vi "包装Main.vi"() -> ()   [LabVIEW 2024]
panel:
  in  "重复包装":dbl
  out "客户码数量":i16
  out "上线码数量":i16
  in  "直接打箱码，慎用！":bool
  out "烘干":bool
  out "烘干工位号":string
  out "重复包装":bool
  in  "切换":bool=TRUE
  in  "扫码结果（流水码）-仅查询":string
  out "清洗":bool
  out "干检":bool
  out "氦检":bool
  out "字符串":string
  out "数值":i32
  out "长度":i32
  out "当前箱码":string
  in  "箱码序号":dbl format="%0#3_5f"
  out "包装完成":bool
  in  "包装累计":dbl
  in  "包装过程":dbl
  in  "扫码结果（客户码）-包装用":string
  in  "设定包装数量":dbl
  in  "装箱产品":string[](array[string])
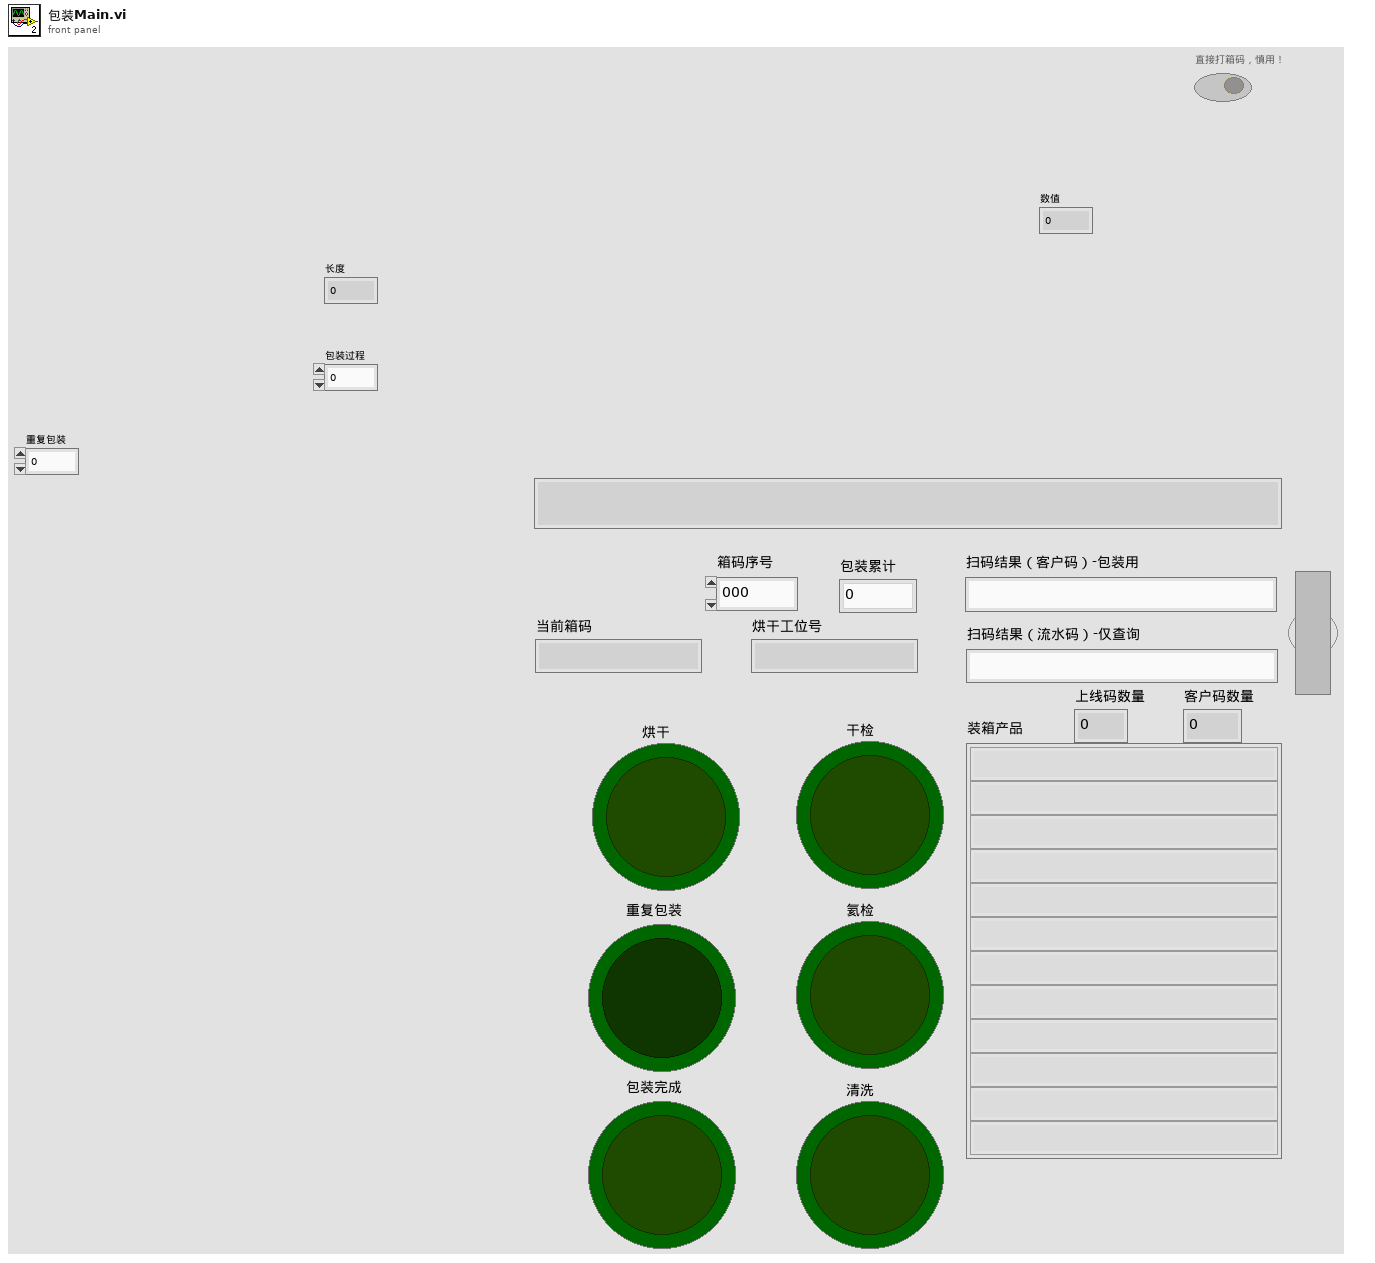
[diagram p1: front panel]
types:
  T1 = enum16{"Standard", "Buffered", "CRLF", "Immediate"}
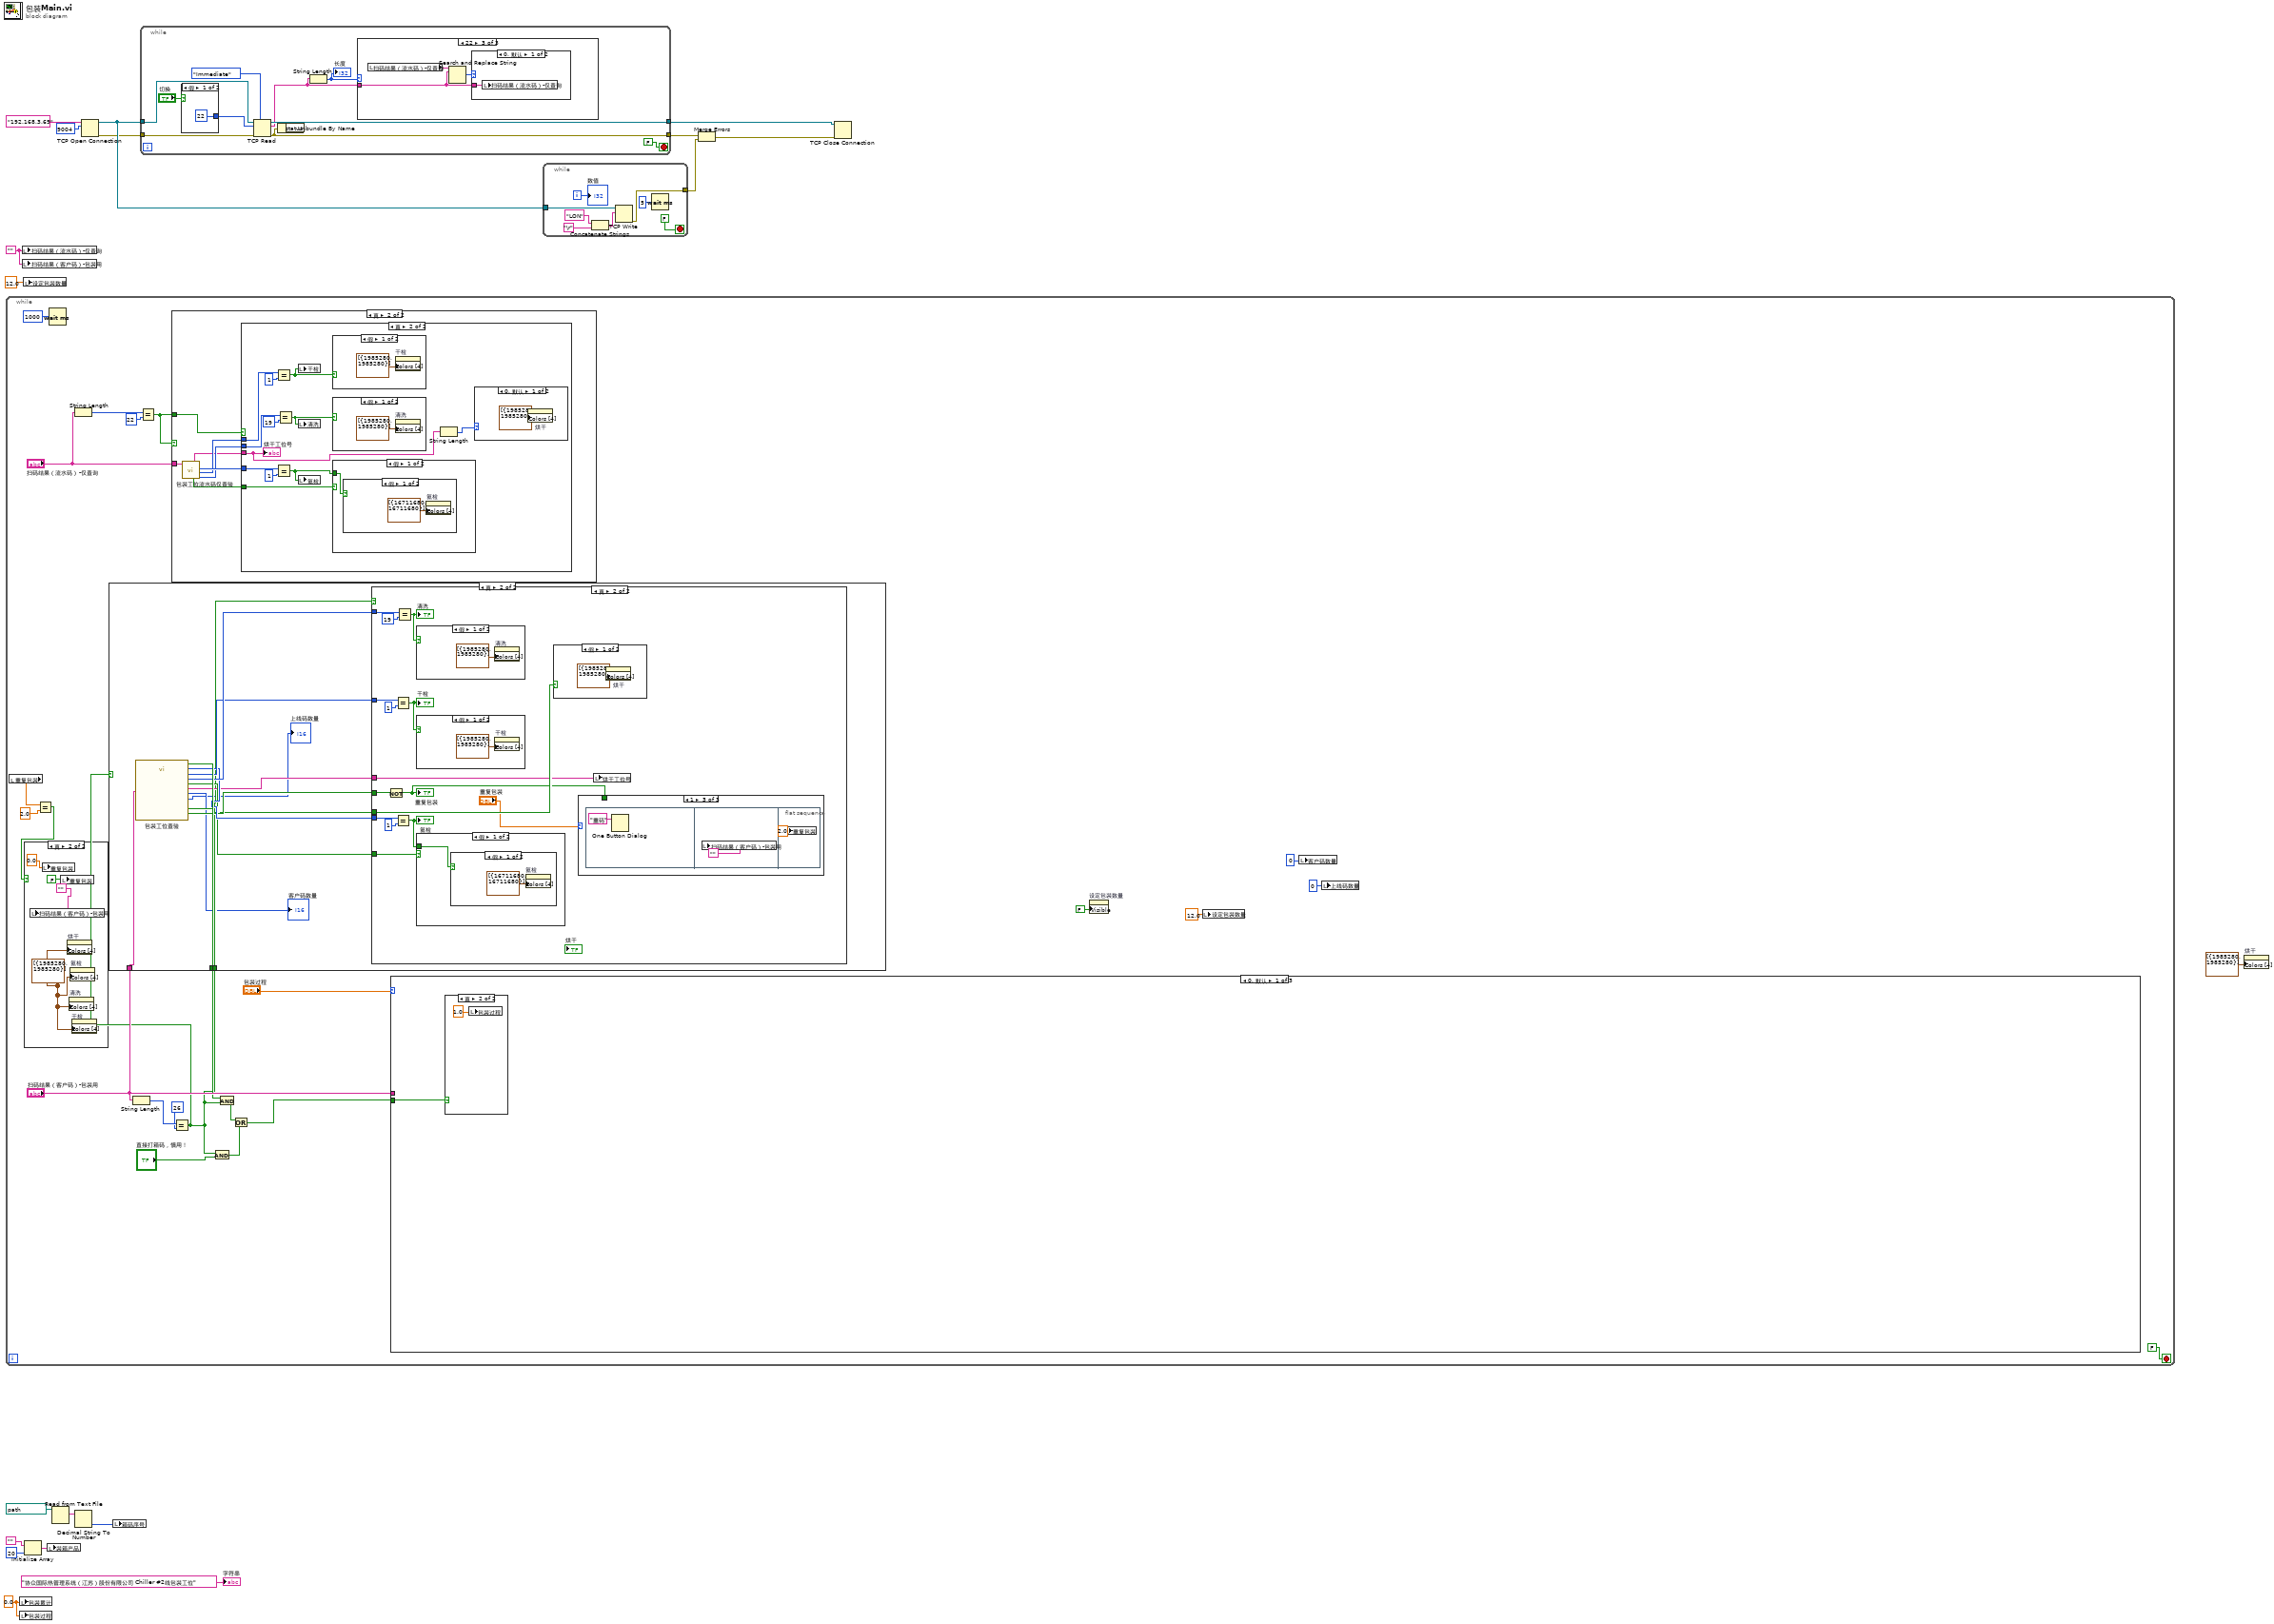
[diagram p0: block diagram]
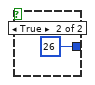
[diagram p2: hidden frame]
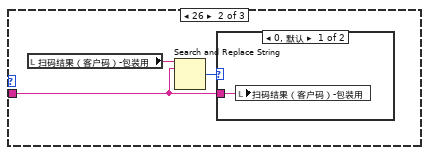
[diagram p4: hidden frame]
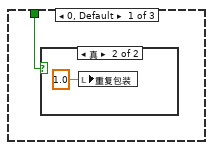
[diagram p10: hidden frame]
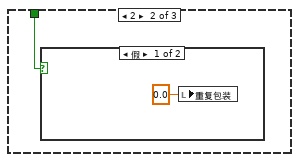
[diagram p12: hidden frame]
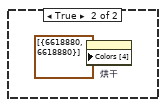
[diagram p14: hidden frame]
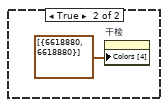
[diagram p15: hidden frame]
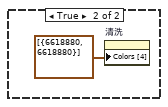
[diagram p16: hidden frame]
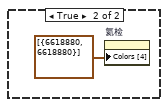
[diagram p17: hidden frame]
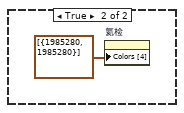
[diagram p18: hidden frame]
diagram:
  w2 = ""
  w19 = 0.0 ("包装过程")
  n1 = while {
    stop <- FALSE stop-if-true
    n2 = local read "重复包装"() -> (w22:dbl)
    n3 = Equal?(x=w22, y=2.0) -> (x = y?=w20:bool)
    n4 = case shown="真" w20 {
      frame False {
      }
      frame True {
        w44 = cluster{u32, u32}[] [{1985280, 1985280}] ("颜色[4]")
        n5 = local write "扫码结果（客户码）-包装用"("") -> ()
        n6 = local write "重复包装"(0.0 ("重复包装")) -> ()
        n7 = local write "重复包装"(FALSE ("重复包装")) -> ()
        n8 = property on="烘干" class="Bool (严格)"("Colors [4]"=w44) -> ()  [unwired: 2 in, 2 out]
        n9 = property on="清洗" class="Bool (严格)"("Colors [4]"=w44) -> ()  [unwired: 2 in, 2 out]
        n10 = property on="氦检" class="Bool (严格)"("Colors [4]"=w44) -> ()  [unwired: 2 in, 2 out]
        n11 = property on="干检" class="Bool (严格)"("Colors [4]"=w44) -> ()  [unwired: 2 in, 2 out]
      }
    }
    n12 = Wait (ms)(milliseconds to wait=u32 1000 ("等待时间（毫秒）")) -> ()  [unwired: 1 out]
    n13 = String Length(string="扫码结果（流水码）-仅查询") -> (length=w34:i32)
    n14 = String Length(string="扫码结果（客户码）-包装用") -> (length=w40:i32)
    n15 = Equal?(x=w34, y=22) -> (x = y?=w28:bool)
    n16 = case shown="真" w28 {
      tunnel: "扫码结果（流水码）-仅查询" -> [_ w97]
      tunnel: w28 -> [_ w96]
      frame False {
      }
      frame True {
        n17 = call "包装工位流水码仅查验.vi"("流水码编号"=w97) -> ("长度"=w93:i32, "干检OK"=w94:i32, "氦检OK"=w95:i32, "没氦检"=w92:bool, "烘干工位号"=w91:string)  [unwired: 5 in, 1 out]
        n18 = case shown="真" w96 {
          tunnel: w95 -> [_ w106]
          tunnel: w94 -> [_ w105]
          tunnel: w93 -> [_ w104]
          tunnel: w92 -> [_ w103]
          tunnel: w91 -> [_ w99]
          frame False {
          }
          frame True {
            n19 = Equal?(x=w105, y=1) -> (x = y?=w100:bool)
            n20 = Equal?(x=w106, y=1) -> (x = y?=w102:bool)
            n21 = Equal?(x=w104, y=19) -> (x = y?=w101:bool)
            n22 = local write "干检"(w100) -> ()
            n23 = local write "清洗"(w101) -> ()
            n24 = local write "氦检"(w102) -> ()
            n25 = case shown="假" w100 {
              frame False {
                n26 = property on="干检" class="Bool (严格)"("Colors [4]"=cluster{u32, u32}[] [{1985280, 1985280}] ("颜色[4]")) -> ()  [unwired: 2 in, 2 out]
              }
              frame True {
                n27 = property on="干检" class="Bool (严格)"("Colors [4]"=cluster{u32, u32}[] [{6618880, 6618880}] ("颜色[4]")) -> ()  [unwired: 2 in, 2 out]
              }
            }
            n28 = case shown="假" w101 {
              frame False {
                n29 = property on="清洗" class="Bool (严格)"("Colors [4]"=cluster{u32, u32}[] [{1985280, 1985280}] ("颜色[4]")) -> ()  [unwired: 2 in, 2 out]
              }
              frame True {
                n30 = property on="清洗" class="Bool (严格)"("Colors [4]"=cluster{u32, u32}[] [{6618880, 6618880}] ("颜色[4]")) -> ()  [unwired: 2 in, 2 out]
              }
            }
            n31 = case shown="假" w103 {
              tunnel: w102 -> [w116 _]
              frame False {
                n32 = case shown="假" w116 {
                  frame False {
                    n33 = property on="氦检" class="Bool (严格)"("Colors [4]"=cluster{u32, u32}[] [{16711680, 16711680}] ("颜色[4]")) -> ()  [unwired: 2 in, 2 out]
                  }
                  frame True {
                    n34 = property on="氦检" class="Bool (严格)"("Colors [4]"=cluster{u32, u32}[] [{6618880, 6618880}] ("颜色[4]")) -> ()  [unwired: 2 in, 2 out]
                  }
                }
              }
              frame True {
                n35 = property on="氦检" class="Bool (严格)"("Colors [4]"=cluster{u32, u32}[] [{1985280, 1985280}] ("颜色[4]")) -> ()  [unwired: 2 in, 2 out]
              }
            }
            n36 = String Length(string=w99) -> (length=w98:i32)
            n37 = case shown="0, 默认" w98 {
              frame 0, Default {
                n38 = property on="烘干" class="Bool (严格)"("Colors [4]"=cluster{u32, u32}[] [{1985280, 1985280}] ("颜色[4]")) -> ()  [unwired: 2 in, 2 out]
              }
              frame 1 {
                n39 = property on="烘干" class="Bool (严格)"("Colors [4]"=cluster{u32, u32}[] [{6618880, 6618880}] ("颜色[4]")) -> ()  [unwired: 2 in, 2 out]
              }
            }
            "烘干工位号" <- w99
          }
        }
      }
    }
    n40 = Equal?(x=w40, y=26) -> (x = y?=w27:bool)
    n41 = case shown="真" w27 {
      tunnel: "扫码结果（客户码）-包装用" -> [_ w58]
      tunnel: [_ w57] -> w37
      tunnel: w27 -> [_ w49]
      frame False {
      }
      frame True {
        n42 = call "包装工位查验.vi"("客户码编号"=w58) -> ("长度"=w56:i32, "干检OK"=w55:i32, "氦检OK"=w54:i32, "可否包装"=w57:bool, "没氦检"=w52:bool, "没包装码"=w53:bool, "烘干工位号"=w50:string, "已经烘干"=w51:bool, "客户码数量"=→"客户码数量":i32, "上线码数量"=→"上线码数量":i32)  [unwired: 1 out]
        n43 = case shown="真" w49 {
          tunnel: w56 -> [_ w70]
          tunnel: w55 -> [_ w69]
          tunnel: w54 -> [_ w68]
          tunnel: w53 -> [_ w67]
          tunnel: w52 -> [_ w66]
          tunnel: w51 -> [_ w62]
          tunnel: w50 -> [_ w61]
          frame False {
          }
          frame True {
            n44 = Not(x=w67) -> (.not. x?=w59:bool)
            "重复包装" <- w59
            n45 = Equal?(x=w69, y=1) -> (x = y?=w64:bool)
            "干检" <- w64
            n46 = Equal?(x=w68, y=1) -> (x = y?=w65:bool)
            "氦检" <- w65
            n47 = Equal?(x=w70, y=19) -> (x = y?=w63:bool)
            "清洗" <- w63
            n48 = case shown="假" w63 {
              frame False {
                n49 = property on="清洗" class="Bool (严格)"("Colors [4]"=cluster{u32, u32}[] [{1985280, 1985280}] ("颜色[4]")) -> ()  [unwired: 2 in, 2 out]
              }
              frame True {
                n50 = property on="清洗" class="Bool (严格)"("Colors [4]"=cluster{u32, u32}[] [{6618880, 6618880}] ("颜色[4]")) -> ()  [unwired: 2 in, 2 out]
              }
            }
            n51 = case shown="假" w64 {
              frame False {
                n52 = property on="干检" class="Bool (严格)"("Colors [4]"=cluster{u32, u32}[] [{1985280, 1985280}] ("颜色[4]")) -> ()  [unwired: 2 in, 2 out]
              }
              frame True {
                n53 = property on="干检" class="Bool (严格)"("Colors [4]"=cluster{u32, u32}[] [{6618880, 6618880}] ("颜色[4]")) -> ()  [unwired: 2 in, 2 out]
              }
            }
            n54 = case shown="假" w66 {
              tunnel: w65 -> [w87 _]
              frame False {
                n55 = case shown="假" w87 {
                  frame False {
                    n56 = property on="氦检" class="Bool (严格)"("Colors [4]"=cluster{u32, u32}[] [{16711680, 16711680}] ("颜色[4]")) -> ()  [unwired: 2 in, 2 out]
                  }
                  frame True {
                    n57 = property on="氦检" class="Bool (严格)"("Colors [4]"=cluster{u32, u32}[] [{6618880, 6618880}] ("颜色[4]")) -> ()  [unwired: 2 in, 2 out]
                  }
                }
              }
              frame True {
                n58 = property on="氦检" class="Bool (严格)"("Colors [4]"=cluster{u32, u32}[] [{1985280, 1985280}] ("颜色[4]")) -> ()  [unwired: 2 in, 2 out]
              }
            }
            n59 = case shown="假" w62 {
              frame False {
                n60 = property on="烘干" class="Bool (严格)"("Colors [4]"=cluster{u32, u32}[] [{1985280, 1985280}] ("颜色[4]")) -> ()  [unwired: 2 in, 2 out]
              }
              frame True {
                n61 = property on="烘干" class="Bool (严格)"("Colors [4]"=cluster{u32, u32}[] [{6618880, 6618880}] ("颜色[4]")) -> ()  [unwired: 2 in, 2 out]
              }
            }
            n62 = case shown="1" "重复包装" {
              tunnel: w59 -> [w74 w76 _]
              frame 0, Default {
                n63 = case shown="真" w74 {
                  frame False {
                  }
                  frame True {
                    n64 = local write "重复包装"(1.0 ("重复包装")) -> ()
                  }
                }
              }
              frame 2 {
                n65 = case shown="假" w76 {
                  frame False {
                    n66 = local write "重复包装"(0.0 ("重复包装")) -> ()
                  }
                  frame True {
                  }
                }
              }
              frame 1 {
                n67 = flat-sequence {
                  frame #0 {
                    n68 = One Button Dialog(message="重码" ("消息")) -> ()  [unwired: 1 in, 1 out]
                  }
                  frame #1 {
                    n69 = local write "扫码结果（客户码）-包装用"("") -> ()
                  }
                  frame #2 {
                    n70 = local write "重复包装"(2.0 ("重复包装")) -> ()
                  }
                }
              }
            }
            n71 = local write "烘干工位号"(w61) -> ()
          }
        }
      }
    }
    n72 = And(x=w27, y="直接打箱码，慎用！") -> (x .and. y?=w29:bool)
    n73 = And(x=w37, y=w27) -> (x .and. y?=w32:bool)
    n74 = Or(x=w32, y=w29) -> (x .or. y?=w31:bool)
    n75 = case shown="0, 默认" "包装过程" {
      tunnel: w31 -> [w120 _ w220]
      tunnel: "扫码结果（客户码）-包装用" -> [_ w128 _]
      frame 0, Default {
        n76 = case shown="真" w120 {
          frame False {
          }
          frame True {
            n77 = local write "包装过程"(1.0 ("包装")) -> ()
          }
        }
      }
      frame 1 {
        n78 = flat-sequence {
          tunnel: w128 -> [w129]
          tunnel: [w129] -> w127
          tunnel: ["设定包装数量"] -> w122
          tunnel: w127 -> [w140]
          tunnel: [w136] -> w126
          tunnel: [w141] -> w123
          tunnel: w122 -> [w141]
          tunnel: w126 -> [w169]
          tunnel: [w169] -> w125
          tunnel: [w168] -> w124
          tunnel: w123 -> [w168]
          tunnel: w125 -> [w171]
          tunnel: w124 -> [w170]
          frame #0 {
            n79 = local read "包装累计"() -> (w131:dbl)
            n80 = case shown="0" w131 {
              frame 0 {
                n81 = Initialize Array("", 20 ("维数大小")) -> (w134:string[])
                n82 = local write "装箱产品"(w134) -> ()
              }
              frame 1, Default {
              }
            }
          }
          frame #1 {
            n83 = flat-sequence {
              tunnel: w140 -> [w143]
              tunnel: ["装箱产品"] -> w139
              tunnel: ["包装累计"] -> w138
              tunnel: [w144] -> w137
              tunnel: [w143] -> w135
              tunnel: w139 -> [w157]
              tunnel: w138 -> [w156]
              tunnel: w137 -> [w158]
              tunnel: [w155] -> w136
              tunnel: w135 -> [w154]
              frame #0 {
                n84 = for {
                  N: "包装累计" -> [_]
                  tunnel: "装箱产品" -> [w153]
                  shift-right: [w147] -> w144
                  shift-left: 0 -> [w149]
                  tunnel: w143 -> [w150]
                  i -> [w152]
                  n85 = Index Array "索引数组"(array=w153, index=w152) -> (element=w151:string)
                  n86 = Search and Replace String "搜索替换字符串"(input string=w151, search string=w150) -> (number of replacements=w148:i32)  [unwired: 6 in, 3 out]
                  n87 = Add(x=w149, y=w148) -> (x+y=w147:i32)
                }
              }
              frame #1 {
                n88 = case shown="0" w158 {
                  tunnel: [w164 _] -> w155
                  tunnel: w157 -> [w163 _]
                  tunnel: w156 -> [w162 _]
                  tunnel: w154 -> [w161 _]
                  frame 0 {
                    n89 = Replace Array Subset "替换数组子集"(array=w163, new element=w161, index=w162) -> (w164:string[])
                    n90 = local read "包装累计"() -> (w160:dbl)
                    n91 = Increment(x=w160) -> (x+1=w159:dbl)
                    n92 = local write "装箱产品"(w164) -> ()
                    n93 = local write "包装累计"(w159) -> ()
                  }
                  frame 1, Default {
                    n94 = local write "扫码结果（客户码）-包装用"("") -> ()
                    n95 = local write "重复包装"(TRUE ("重复包装")) -> ()
                    n96 = One Button Dialog(message="重码" ("消息")) -> ()  [unwired: 1 in, 1 out]
                  }
                }
              }
            }
          }
          frame #2 {
          }
          frame #3 {
            n97 = local read "包装累计"() -> (w172:dbl)
            n98 = Equal?(x=w170, y=w172) -> (x = y?=w173:bool)
            n99 = case shown="真" w173 {
              tunnel: w172 -> [_ w176]
              tunnel: w171 -> [_ w175]
              frame False {
                n100 = local write "包装完成"(FALSE ("包装")) -> ()
              }
              frame True {
                n101 = flat-sequence {
                  tunnel: w176 -> [w179]
                  tunnel: w175 -> [w178]
                  frame #0 {
                    n102 = for {
                      N: w179 -> [w181]
                      tunnel: w178 -> [w201]
                      i -> [w189]
                      n103 = local read "箱码序号"() -> (w199:dbl)
                      n104 = Number To Decimal String(number=w181) -> (decimal integer string=w180:string)  [unwired: 1 in]
                      n105 = Number To Decimal String(number=w189) -> (decimal integer string=w186:string)  [unwired: 1 in]
                      n106 = Write to Text File(file (use dialog)=path "D:/数量.txt" ("文件（使用对话框）"), text=w180) -> ()  [unwired: 2 in, 3 out]
                      n107 = Number To Decimal String(number=w199, width (-)=i16 3 ("宽度(-)")) -> (decimal integer string=w198:string)
                      n108 = Concatenate Strings("D:\\装箱激光码" ("时间格式字符串(%c)"), w186, ".txt" ("时间格式字符串(%c)")) -> (w185:string)
                      n109 = call <vilib>:"Space Constant.vi"() -> ("String"=w197:string)
                      n110 = Search and Replace String(replace all?=TRUE ("替换全部？(F)"), input string=w198, search string=w197, replace string="0" ("替换字符串(\"\")")) -> (result string=w192:string)  [unwired: 4 in, 3 out]
                      n111 = String To Path(string=w185) -> (path=w184:path)
                      n112 = Format Date/Time String(time format string (%c)="%Y%m%d" ("时间格式字符串(%c)")) -> (date/time string=w193:string)  [unwired: 2 in]
                      n113 = Index Array(array=w201, index=w189) -> (element=w183:string)
                      n114 = Concatenate Strings(w193, w192) -> (w191:string)
                      "当前箱码" <- w191
                      n115 = Write to Text File(file (use dialog)=w184, text=w183) -> ()  [unwired: 2 in, 3 out]
                      n116 = Write to Text File(file (use dialog)=path "D:/最终装箱码.txt" ("文件（使用对话框）"), text=w191) -> ()  [unwired: 2 in, 3 out]
                      n117 = call "数据库包装标记更新.vi"("激光码信息"=w183, "箱码"=w191) -> ()  [unwired: 10 in]
                    }
                  }
                  frame #1 {
                    n118 = Wait (ms)(milliseconds to wait=u32 1500 ("等待时间（毫秒）")) -> ()  [unwired: 1 out]
                  }
                  frame #2 {
                    n119 = call "Bartender打印子vi.vi"() -> ()  [unwired: 12 in]
                    n120 = Increment(x="箱码序号") -> (x+1=w205:dbl)
                    n121 = local write "箱码序号"(w205) -> ()
                    n122 = Number To Decimal String(number=w205) -> (decimal integer string=w204:string)  [unwired: 1 in]
                    n123 = Write to Text File(file (use dialog)=path "D:/箱码.txt" ("文件（使用对话框）"), text=w204) -> ()  [unwired: 2 in, 3 out]
                  }
                  frame #3 {
                    n124 = Wait (ms)(milliseconds to wait=u32 1500 ("等待时间（毫秒）")) -> ()  [unwired: 1 out]
                  }
                }
                n125 = flat-sequence {
                  frame #0 {
                    "包装完成" <- TRUE ("包装")
                  }
                  frame #1 {
                    n126 = Wait (ms)(milliseconds to wait=u32 1000 ("等待时间（毫秒）")) -> ()  [unwired: 1 out]
                  }
                  frame #2 {
                    n127 = local write "包装完成"(FALSE ("包装")) -> ()
                  }
                }
                n128 = local write "包装累计"(0.0 ("包装累计")) -> ()
              }
            }
          }
          frame #4 {
            n129 = Wait (ms)(milliseconds to wait=u32 1500 ("等待时间（毫秒）")) -> ()  [unwired: 1 out]
          }
          frame #5 {
            w217 = ""
            n130 = local write "扫码结果（客户码）-包装用"(w217) -> ()
            n131 = local write "扫码结果（流水码）-仅查询"(w217) -> ()
            n132 = property on="清洗" class="Bool (严格)"("Colors [4]"=cluster{u32, u32}[] [{1985280, 1985280}] ("颜色[4]")) -> ()  [unwired: 2 in, 2 out]
            n133 = property on="干检" class="Bool (严格)"("Colors [4]"=cluster{u32, u32}[] [{1985280, 1985280}] ("颜色[4]")) -> ()  [unwired: 2 in, 2 out]
            n134 = property on="氦检" class="Bool (严格)"("Colors [4]"=cluster{u32, u32}[] [{1985280, 1985280}] ("颜色[4]")) -> ()  [unwired: 2 in, 2 out]
            n135 = local write "客户码数量"(i16 0 ("客户码数量")) -> ()
            n136 = property on="烘干" class="Bool (严格)"("Colors [4]"=cluster{u32, u32}[] [{1985280, 1985280}] ("颜色[4]")) -> ()  [unwired: 2 in, 2 out]
            n137 = local write "上线码数量"(i16 0 ("上线码数量")) -> ()
          }
          frame #6 {
            n138 = local write "包装过程"(2.0 ("包装过程")) -> ()
          }
        }
      }
      frame 2 {
        n139 = case shown="假" w220 {
          frame False {
            n140 = local write "包装过程"(0.0 ("包装过程")) -> ()
          }
          frame True {
          }
        }
      }
    }
    n141 = property on="设定包装数量" class="DigNum (严格)"("Visible"=FALSE ("可见")) -> ()  [unwired: 2 in, 2 out]
    n142 = local write "设定包装数量"(12.0 ("设定包装数量")) -> ()
    n143 = local write "客户码数量"(i16 0 ("客户码数量")) -> ()
    n144 = local write "上线码数量"(i16 0 ("上线码数量")) -> ()
  }
  n145 = local write "包装累计"(w19) -> ()
  n146 = local write "包装过程"(w19) -> ()
  n147 = local write "扫码结果（流水码）-仅查询"(w2) -> ()
  n148 = local write "扫码结果（客户码）-包装用"(w2) -> ()
  n149 = local write "设定包装数量"(12.0 ("设定包装数量")) -> ()
  n150 = Initialize Array("", 20 ("维数大小")) -> (w16:string[])
  n151 = local write "装箱产品"(w16) -> ()
  n152 = Read from Text File(file (use dialog)=path "D:/箱码.txt" ("文件（使用对话框）")) -> (text=w14:string)  [unwired: 3 in, 3 out]
  n153 = Decimal String To Number(string=w14) -> (number=w13:i32)  [unwired: 2 in, 1 out]
  n154 = TCP Open Connection(address="192.168.3.69" ("地址"), remote port or service name=u16 9004 ("远程端口或服务名称")) -> (connection ID=w10:refnum<k5>, error out=w9:errorcluster)  [unwired: 3 in]
  n155 = local write "箱码序号"(w13) -> ()
  n156 = while {
    tunnel: w10 -> [w231]
    tunnel: w9 -> [w230]
    tunnel: [w228] -> w11
    tunnel: [w227] -> w6
    stop <- FALSE stop-if-true
    n157 = case shown="假" "切换" {
      tunnel: [22 ("读取的字节") 26 ("读取的字节")] -> w226
      frame False {
      }
      frame True {
      }
    }
    n158 = TCP Read(connection ID=w231, bytes to read=w226, error in (no error)=w230, 7:T1."Immediate" ("模式（标准）")) -> (connection ID out=w228:refnum<k5>, data out=w224:string, error out=w227:errorcluster)  [unwired: 1 in]
    n159 = Unbundle By Name(w227) -> ()  [unwired: 1 out]
    n160 = String Length(string=w224) -> (length=w225:i32)
    "长度" <- w225
    n161 = case shown="22" w225 {
      tunnel: w224 -> [_ w234 w238]
      frame 0, Default {
      }
      frame 26 {
        n162 = local read "扫码结果（客户码）-包装用"() -> (w236:string)
        n163 = Search and Replace String(input string=w236, search string=w234) -> (number of replacements=w235:i32)  [unwired: 6 in, 3 out]
        n164 = case shown="0, 默认" w235 {
          tunnel: w234 -> [w237 _]
          frame 0, Default {
            n165 = local write "扫码结果（客户码）-包装用"(w237) -> ()
          }
          frame 1 {
          }
        }
      }
      frame 22 {
        n166 = local read "扫码结果（流水码）-仅查询"() -> (w240:string)
        n167 = Search and Replace String(input string=w240, search string=w238) -> (number of replacements=w239:i32)  [unwired: 6 in, 3 out]
        n168 = case shown="0, 默认" w239 {
          tunnel: w238 -> [w241 _]
          frame 0, Default {
            n169 = local write "扫码结果（流水码）-仅查询"(w241) -> ()
          }
          frame 1 {
          }
        }
      }
    }
  }
  n170 = while {
    tunnel: w10 -> [w249]
    tunnel: [w248] -> w5
    i -> [w242]
    stop <- FALSE stop-if-true
    n171 = Concatenate Strings("LON" ("数据输入"), "\r") -> (w243:string)
    n172 = TCP Write(connection ID=w249, data in=w243) -> (error out=w248:errorcluster)  [unwired: 2 in, 2 out]
    n173 = Wait (ms) ("等待(ms)")(milliseconds to wait=u32 5 ("等待时间（毫秒）")) -> ()  [unwired: 1 out]
    "数值" <- w242
  }
  n174 = Merge Errors(w6, w5) -> (w12:errorcluster)
  n175 = TCP Close Connection(connection ID=w11, error in (no error)=w12) -> ()  [unwired: 1 in, 2 out]
  n176 = property on="烘干" class="Bool (严格)"("Colors [4]"=cluster{u32, u32}[] [{1985280, 1985280}] ("颜色[4]")) -> ()  [unwired: 2 in, 2 out]
  "字符串" <- "协众国际热管理系统（江苏）股份有限公司 Chiller #2线包装工位" ("字符串")
